vi "Check ECAT Installed.vi"(8 "error in":errorcluster) -> (0 "error out":errorcluster)   [LabVIEW 2020, in "SEECD System Explorer.lvlib"]
uses:
  SEECD System Explorer.lvlib
  <vilib>/registry/registry.llb/Registry RtKey.ctl
  <vilib>/registry/registry.llb/Registry SAM.ctl
  <vilib>/registry/registry.llb/Read Registry Value Simple STR.vi
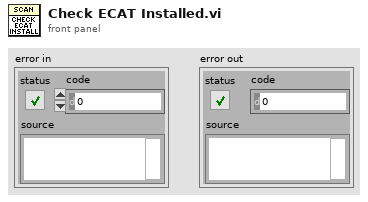
[diagram p1: front panel]
types:
  T1 = typedef "Registry SAM.ctl" = enum32{"KEY_QUERY_VALUE", "KEY_SET_VALUE", "KEY_CREATE_SUB_KEY", "KEY_ENUMERATE_SUB_KEYS", "KEY_NOTIFY", "KEY_CREATE_LINK", "KEY_READ", "KEY_WRITE", "KEY_ALL_ACCESS", "KEY_READ | KEY_WRITE"}
  T2 = typedef "Registry RtKey.ctl" = enum32{"HKEY_CLASSES_ROOT", "HKEY_CURRENT_USER", "HKEY_LOCAL_MACHINE", "HKEY_USERS", "HKEY_PERFORMANCE_DATA", "HKEY_CURRENT_CONFIG", "HKEY_DYN_DATA"}
  T3 = typedef "Registry refnum.ctl" = refnum<k1>
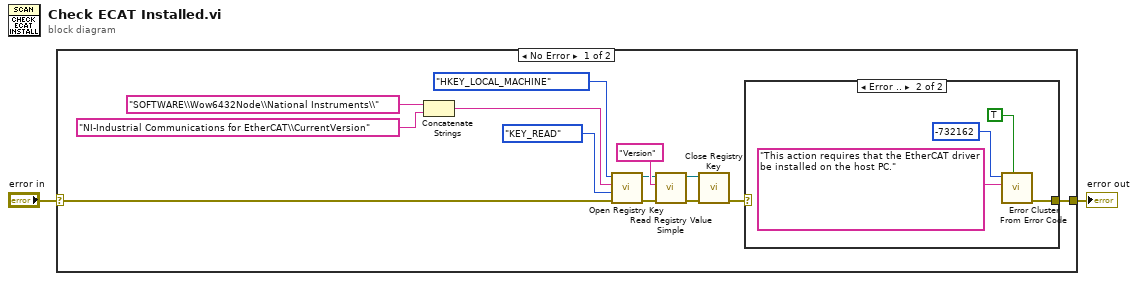
[diagram p0: block diagram]
diagram:
  n1 = case shown="No Error" "error in" {
    selector: "error in" -> [w3 w21]
    tunnel: [w7 w21] -> w2
    frame No Error {
      n2 = Concatenate Strings("SOFTWARE\\Wow6432Node\\National Instruments\\", "NI-Industrial Communications for EtherCAT\\CurrentVersion") -> (w15:string)
      n3 = call <vilib>:"Open Registry Key.vi"("error in (no error)"=w3, "security access mask (KEY_READ | KEY_WRITE)"=Registry_SAM."KEY_READ", "subkey"=w15, "root key (HKEY_LOCAL_MACHINE)"=Registry_RtKey."HKEY_LOCAL_MACHINE") -> ("error out"=w12:errorcluster, "refnum out"=w13:T3)  [unwired: 6 in]
      n4 = call-poly <vilib>:"Read Registry Value Simple.vi"("error in (no error)"=w12, "value"="Version", "refnum"=w13) -> ("error out"=w8:errorcluster, "refnum out"=w9:T3)  [unwired: 3 in, 2 out]
      n5 = call <vilib>:"Close Registry Key.vi"("error in (no error)"=w8, "refnum"=w9) -> ("error out"=w6:errorcluster)  [unwired: 5 in]
      n6 = case shown="Error .." w6 {
        selector: w6 -> [w16 _]
        tunnel: [w16 w17] -> w7
        frame No Error {
        }
        frame Error {
          n7 = call <vilib>:"Error Cluster From Error Code.vi"("show call chain? (False)"=TRUE, "error message (\"\")"="This action requires that the EtherCAT driver be installed on the host PC." ("error message (\"\")"), "error code (0)"=-732162) -> ("error out"=w17:errorcluster)  [unwired: 6 in]
        }
      }
    }
    frame Error {
    }
  }
  "error out" <- w2
